vi "populate_io_index_array.vi"(8 "error in (no error)":errorcluster, 11 "IO_variables_per_module":T1) -> (0 "error out":errorcluster, 3 "IO_table_index_ordered":i32[](array[numeric]))   [LabVIEW 2015, in "Scan Engine runtime.lvclass"]
uses:
  Scan Engine runtime.lvclass
  Custom Ctrls/IO_index_map.ctl
  <vilib>/NI/Tag Bus/tag/Data Type.ctl
  Custom Ctrls/Index Map.ctl
  <resource>/objmgr/ni.var.rc
  <vilib>/NI/Tag Bus/tag/tag descriptor.lvclass
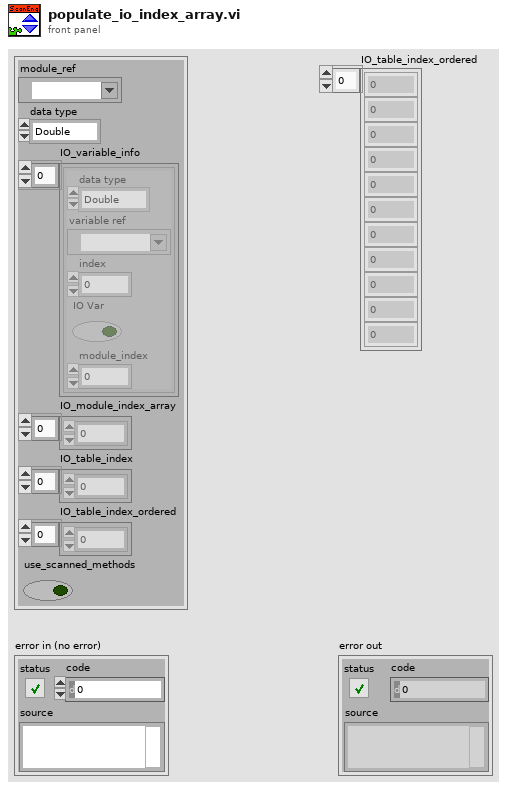
[diagram p1: front panel]
types:
  T1 = typedef "Scan Engine runtime.lvclass/IO_index_map.ctl" = cluster{"module_ref":refnum<k21>, "data type":T2, "IO_variable_info":T3[], "IO_module_index_array":i32[], "IO_table_index":i32[], "IO_table_index_ordered":i32[], "use_scanned_methods":bool}
  T2 = typedef "tag bus.lvlib/tag descriptor.lvclass/Data Type.ctl" = enum16{"Double", "Single", "I64", "I32", "I16", "I8", "U64", "U32", "U16", "U8", "Boolean", "String", "Array of Double", "Array of Single", "Array of I64", "Array of I32", "Array of I16", "Array of I8", "Array of U64", "Array of U32", "Array of U16", "Array of U8", "Array of Boolean", "Array of String"}
  T3 = typedef "Scan Engine runtime.lvclass/Index Map.ctl" = cluster{"data type":T2, "variable ref":refnum<k21>, "index":i32, "IO Var":bool, "module_index":i32}
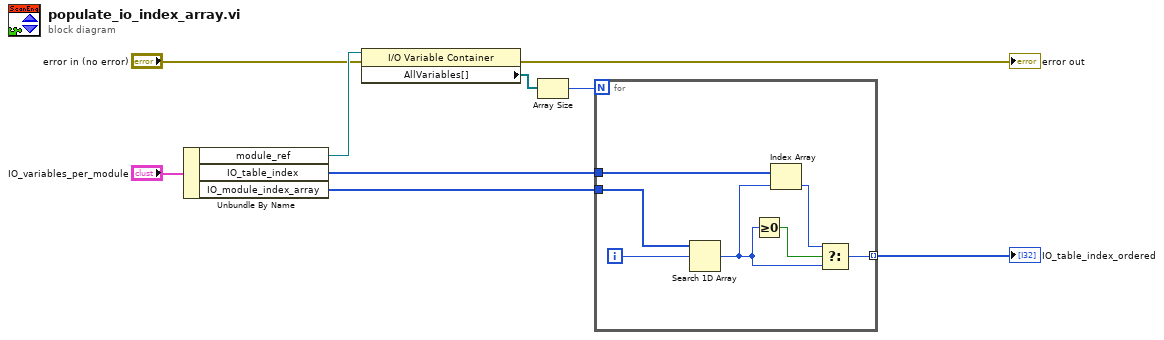
[diagram p0: block diagram]
diagram:
  n1 = Unbundle By Name("IO_variables_per_module") -> ("module_ref"=w4:refnum<k21>, "IO_table_index"=w7:i32[], "IO_module_index_array"=w8:i32[])
  n2 = property class="I/O Variable Container"(reference=w4, error in="error in (no error)") -> (error out=→"error out":errorcluster, "AllVariables[]"=w6:refnum<k21>[])  [unwired: 1 out]
  n3 = Array Size(array=w6) -> (size(s)=w5:i32)
  n4 = for {
    N: w5 -> [_]
    tunnel: w8 -> [w16]
    tunnel: w7 -> [w14]
    tunnel: [w12] -> w3 mode=indexing
    i -> [w15]
    n5 = Search 1D Array(1D array=w16, element=w15) -> (index of element=w10:i32)  [unwired: 1 in]
    n6 = Greater Or Equal To 0?(x=w10) -> (x >= 0?=w11:bool)
    n7 = Index Array(array=w14, index=w10) -> (element=w13:i32)
    n8 = Select(t=w13, s=w11, f=w10) -> (s? t:f=w12:i32)
  }
  "IO_table_index_ordered" <- w3
